vi "Handle Error.vi"(8 "error in (no error)":errorcluster, 11 "ZM-HWM-hardware_manager in":refnum<class "ZM-HWM-hardware_manager.lvclass">) -> (0 "error out":errorcluster, 2 "stop actor?":bool=TRUE, 3 "ZM-HWM-hardware_manager out":refnum<class "ZM-HWM-hardware_manager.lvclass">)   [LabVIEW 2020, in "ZM-HWM-hardware_manager.lvlib" / "ZM-HWM-hardware_manager.lvclass"]
doc: "Handle Error override of the hardware manager: Call Parent first (it clears error 43 from a normal stop), then ZM-HWM-evaluateError. Error-handling plan: none yet; evaluateError passes the error on, so an error stops the hardware manager and, through its Last Ack, its caller."
uses:
  ZM-HWM-hardware_manager.lvclass
  <vilib>/ActorFramework/Actor/Actor.lvclass
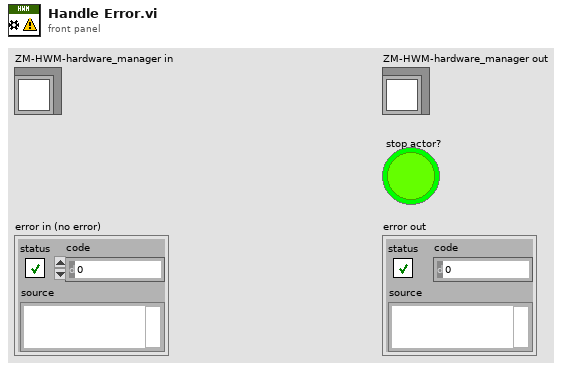
[diagram p1: front panel]
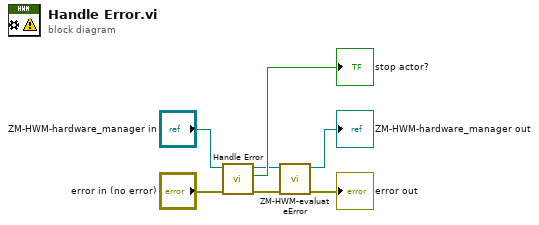
[diagram p0: block diagram]
diagram:
  n1 = call-parent "Handle Error.vi"("error in (no error)"="error in (no error)", "Actor in"="ZM-HWM-hardware_manager in") -> ("error out"=w1:errorcluster, "stop actor?"=→"stop actor?":bool, "Actor out"=w3:refnum<class "ZM-HWM-hardware_manager.lvclass">)  [unwired: 7 in]
  n2 = call "ZM-HWM-evaluateError.vi"("error in (no error)"=w1, "ZM-HWM-hardware_manager in"=w3) -> ("error out"=→"error out":errorcluster, "ZM-HWM-hardware_manager out"=→"ZM-HWM-hardware_manager out":refnum<class "ZM-HWM-hardware_manager.lvclass">)  [unwired: 7 in, 1 out]
